vi "Check Deviation Attributes.vi"(8 "error in (no error)":errorcluster, 11 "Deviation In":string) -> (0 "error out":errorcluster, 3 "Deviation Out":string)   [LabVIEW 2019, in "Path Settings.lvclass"]
uses:
  Path Settings.lvclass
  subVIs/typedefs/Schedule Types/Schedule--Formula.ctl
  <vilib>/JDP Science/JSONtext/Next JSON Value.vi
  <vilib>/JDP Science/JSONtext/String Subset.vi
  <vilib>/JDP Science/JSONtext/Parsing/Advance past next JSON Value (inlined COPY).vi
  <vilib>/JDP Science/JSONtext/Parsing/Advance past whitespace.vi
  <vilib>/JDP Science/JSONtext/Parsing/Advance past String.vi
  <vilib>/JDP Science/JSONtext/Parsing/Advance past Number.vi
  <vilib>/JDP Science/JSONtext/Parsing/Advance past Line Ending.vi
  <vilib>/JDP Science/JSONtext/Parsing/Parse Full Path or Item Name.vi
  <vilib>/JDP Science/JSONtext/Parsing/Advance past Array.vi
  <vilib>/JDP Science/JSONtext/Parsing/Advance past Object.vi
  <vilib>/JDP Science/JSONtext/support/Error Cluster From Code.vi
  <vilib>/JDP Science/JSONtext/Offset/Find Item Locations by Path.vi
  ObjectSettings/ObjectSettings.lvclass
  <vilib>/JDP Science/JSONtext/JSONtext.lvlib
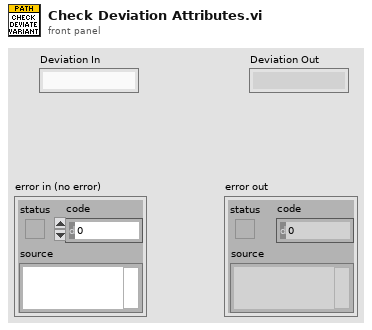
[diagram p1: front panel]
types:
  T1 = typedef "Schedule--Formula.ctl" = cluster{"formula":string, "formula length (nm)":dbl, "formula resolution (nm)":dbl}
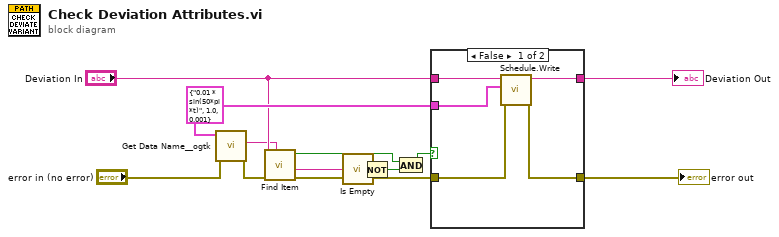
[diagram p0: block diagram]
diagram:
  w13 = T1 {"formula"="0.01 * sin(50*pi*t)", "formula length (nm)"=1.0, "formula resolution (nm)"=0.001} ("Formula")
  n1 = call <userlib>:"Get Data Name__ogtk.vi"("error in (no error)"="error in (no error)", "Data"=w13) -> ("error out"=w8:errorcluster, "Data Name"=w6:string)  [unwired: 7 in, 1 out]
  n2 = call <vilib>:"Find Item.vi"("$Path or Item Name"=w6, "error in (no error)"=w8, "JSON"="Deviation In") -> ("error out"=w9:errorcluster, "<JSON>"=w5:string, "Found"=w3:bool)  [unwired: 5 in, 1 out]
  n3 = call <vilib>:"Is Empty.vi"("JSON"=w5) -> ("Empty"=w4:bool)  [unwired: 4 in]
  n4 = Not(x=w4) -> (.not. x?=w1:bool)
  n5 = And(x=w3, y=w1) -> (x .and. y?=w2:bool)
  n6 = case shown="False" w2 {
    tunnel: w13 -> [w18 _]
    tunnel: "Deviation In" -> [w17 w20]
    tunnel: [w16 w20] -> w10
    tunnel: [w15 w19] -> w11
    tunnel: w9 -> [w14 w19]
    frame False {
      n7 = call "Schedule.Write.vi"("error in (no error)"=w14, "Data to Write"=w18, "Schedule <JSON> In"=w17) -> ("error out"=w15:errorcluster, "Schedule <JSON> Out"=w16:string)  [unwired: 7 in]
    }
    frame True {
    }
  }
  "error out" <- w11
  "Deviation Out" <- w10
